vi "DSS-test-lin_calc_impedance2.vi"(8 "error in":errorcluster) -> (0 "error out":errorcluster)   [LabVIEW 2020, in "DSS-Tests.lvlib"]
doc: "Caraya test of RDC-Lin-Calc_Impedance2 on a four-point Common Format (1e8 to 6e9 Hz, reflections 0, 0.5, -0.5, 0.3+0.4i, all other arrays zero): Output cluster and Impedance against their golden file."
uses:
  DSS-Tests.lvlib
  <vilib>/addons/_JKI Toolkits/Caraya/classes/Test/Test.lvclass
  Computation/RDC-Reflection_Data_Computation.lvlib
  <vilib>/addons/_JKI Toolkits/Caraya/classes/Assert/Assert.lvclass
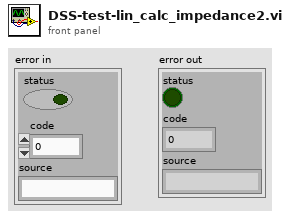
[diagram p1: front panel]
types:
  T1 = cluster{"Frequency":dbl[], "Reflection'":dbl[], "Reflection''":dbl[], "Permativity'":dbl[], "Permativity''":dbl[], "Conductivity":dbl[], "Loss Tangent":dbl[], "Resistance":dbl[], "Reactance":dbl[]}
  T2 = typedef "RFH-Reflection_File_Handler.lvlib/RFH-common_data_format.ctl" = cluster{"Frequency":dbl[], "Reflection'":dbl[], "Reflection''":dbl[], "Permativity'":dbl[], "Permativity''":dbl[], "Conductivity":dbl[], "Loss Tangent":dbl[], "Resistance":dbl[], "Reactance":dbl[]}
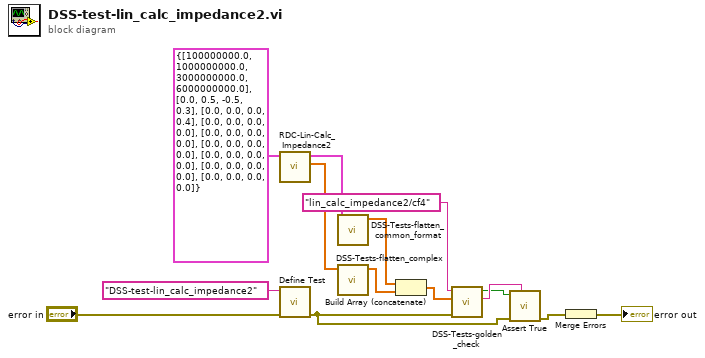
[diagram p0: block diagram]
diagram:
  n1 = call "RDC-Lin-Calc_Impedance2.vi"("input cluster"=T1 {"Frequency"=[100000000.0, 1000000000.0, 3000000000.0, 6000000000.0], "Reflection'"=[0.0, 0.5, -0.5, 0.3], "Reflection''"=[0.0, 0.0, 0.0, 0.4], "Permativity'"=[0.0, 0.0, 0.0, 0.0], "Permativity''"=[0.0, 0.0, 0.0, 0.0], "Conductivity"=[0.0, 0.0, 0.0, 0.0], "Loss Tangent"=[0.0, 0.0, 0.0, 0.0], "Resistance"=[0.0, 0.0, 0.0, 0.0], "Reactance"=[0.0, 0.0, 0.0, 0.0]}) -> ("Impedance"=w6:cdb[], "Output cluster"=w5:T2)  [unwired: 9 in]
  n2 = call <vilib>:"Define Test.vi"("error in (no error)"="error in", "Label (VI Title)"="DSS-test-lin_calc_impedance2") -> ("error out"=w3:errorcluster)  [unwired: 8 in, 1 out]
  n3 = call "DSS-Tests-flatten_common_format.vi"("Common Format"=w5) -> ("flat"=w7:dbl[])  [unwired: 10 in]
  n4 = call "DSS-Tests-flatten_complex.vi"("values"=w6) -> ("flat"=w8:dbl[])  [unwired: 10 in]
  n5 = Build Array (concatenate)(w7, w8) -> (w9:dbl[])
  n6 = call "DSS-Tests-golden_check.vi"("error in"=w3, "actual"=w9, "golden name"="lin_calc_impedance2/cf4") -> ("message"=w12:string, "pass"=w11:bool)  [unwired: 6 in, 1 out]
  n7 = call <vilib>:"Assert True.vi"("Label"=w12, "error in (no error)"=w3, "True?"=w11) -> ("error out"=w13:errorcluster)  [unwired: 7 in, 1 out]
  n8 = Merge Errors(w13) -> (→"error out":errorcluster)
